vi "CANsub_Codec_LibPath.vi"() -> (3 "Path":path=path "/usr/local/lib/libcansub_codec.*")   [LabVIEW 2021, in "CANsub_Codec.lvlib"]
uses:
  CANsub_Codec.lvlib
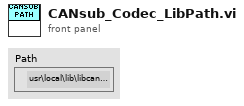
[diagram p1: front panel]
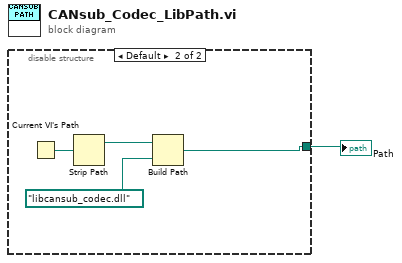
[diagram p0: block diagram]
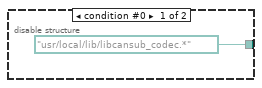
[diagram p2: hidden frame]
diagram:
  n1 = disable-structure shown="Default" {
    disable-tunnel: [path "/usr/local/lib/libcansub_codec.*" w3] -> w1
    frame condition #0 {
    }
    frame condition #1 (active) {
      n2 = Current VI's Path() -> (path=w6:path)
      n3 = Strip Path(path=w6) -> (stripped path=w5:path)  [unwired: 1 out]
      n4 = Build Path(base path=w5, name or relative path=path "libcansub_codec.dll") -> (appended path=w3:path)
    }
  }
  "Path" <- w1
